vi "Refresh Scroll.vi"(8 "error in (no error)":errorcluster, 11 "2DArrayManager in":refnum<class "2DArrayManager.lvclass">) -> (0 "error out":errorcluster, 3 "2DArrayManager out":refnum<class "2DArrayManager.lvclass">)   [LabVIEW 2020, in "OOPanel.lvlib" / "2DArrayManager.lvclass"]
uses:
  2DArrayManager.lvclass
  2DArrayManager.lvclass/2DArrayManager.ctl
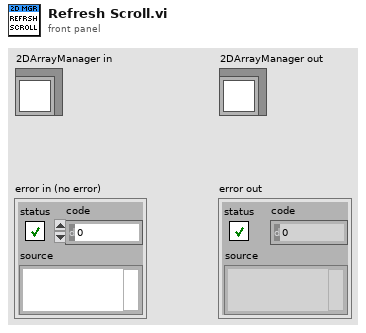
[diagram p1: front panel]
types:
  T1 = typedef "OOPanel.lvlib/2DArrayManager.lvclass/Options.ctl" = cluster{"Running":bool, "Borders":bool, "Background":u32, "V Scroll":bool, "H Scroll":bool, "Blank":refnum<class "2DPanelBlank.lvclass">, "Initial Blank Count":i32}
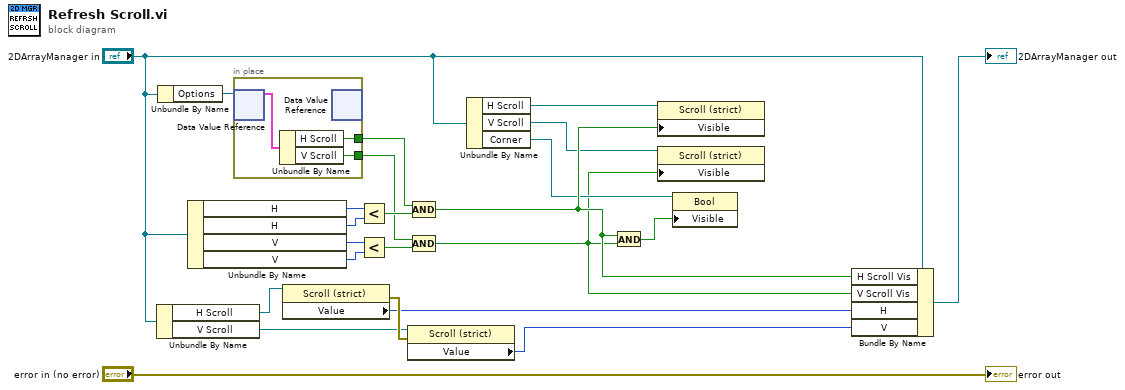
[diagram p0: block diagram]
diagram:
  n1 = Unbundle By Name("2DArrayManager in") -> ("H Scroll"=w21:refnum<vi>, "V Scroll"=w20:refnum<vi>)
  n2 = Unbundle By Name("2DArrayManager in") -> ("Options"=w18:refnum<data-value>)
  n3 = Unbundle By Name("2DArrayManager in") -> ("H"=w15:i32, "H"=w14:i32, "V"=w13:i32, "V"=w12:i32)
  n4 = in-place {
    in-place-border: [w25] -> w9
    in-place-border: [w24] -> w8
    n5 = in-place-dvr #1(w18) -> (w26:T1)  [unwired: 1 out]
    n6 = Unbundle By Name(w26) -> ("H Scroll"=w25:bool, "V Scroll"=w24:bool)
    n7 = in-place-dvr #1() -> ()  [unwired: 1 in, 2 out]
  }
  n8 = property class="Scroll (strict)"(reference=w21) -> (error out=w23:errorcluster, "Value"=w17:i32)  [unwired: 1 in, 1 out]
  n9 = Less?(x=w15, y=w14) -> (x < y?=w11:bool)
  n10 = Less?(x=w13, y=w12) -> (x < y?=w10:bool)
  n11 = property class="Scroll (strict)"(reference=w20, error in=w23) -> ("Value"=w16:i32)  [unwired: 2 out]
  n12 = Compound Arithmetic op=AND(w9, w11) -> (w5:bool)
  n13 = Compound Arithmetic op=AND(w8, w10) -> (w1:bool)
  n14 = Unbundle By Name("2DArrayManager in") -> ("H Scroll"=w6:refnum<vi>, "V Scroll"=w2:refnum<vi>, "Corner"=w3:refnum<vi>)
  n15 = And(x=w5, y=w1) -> (x .and. y?=w4:bool)
  n16 = property class="Scroll (strict)"(reference=w6, "Visible"=w5) -> ()  [unwired: 1 in, 2 out]
  n17 = property class="Scroll (strict)"(reference=w2, "Visible"=w1) -> ()  [unwired: 1 in, 2 out]
  n18 = property class="Bool"(reference=w3, "Visible"=w4) -> ()  [unwired: 1 in, 2 out]
  n19 = Bundle By Name(cluster="2DArrayManager in", "H Scroll Vis"=w5, "V Scroll Vis"=w1, "H"=w17, "V"=w16) -> (→"2DArrayManager out":refnum<class "2DArrayManager.lvclass">)
  "error out" <- "error in (no error)"
